vi "gdi32 DeleteObject.vi"(0 "ho":u64, 11 "error in":errorcluster) -> (4 "return value":i32, 15 "error out":errorcluster)   [LabVIEW 2020, in "RemoteVI.lvlib"]
doc: "Deletes a GDI object (bitmap, pen, brush ...) through gdi32.dll DeleteObject (stdcall, called in any thread). It must not be selected into a device context. return value is non-zero on success. When error in carries an error the DLL is not called. Generated by scripts\\Build Win32 Wrappers.vi - do not edit by hand, rebuild it."
uses:
  RemoteVI.lvlib
  gdi32.dll
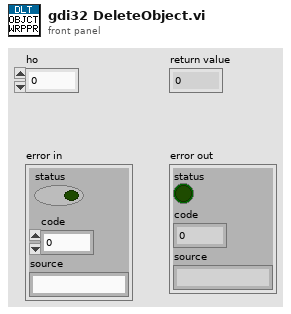
[diagram p1: front panel]
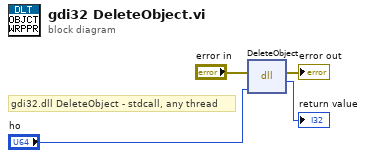
[diagram p0: block diagram]
diagram:
  # "gdi32.dll DeleteObject - stdcall, any thread"
  n1 = dll-call lib="gdi32.dll" fn="DeleteObject"(error in="error in", "ho"="ho") -> (error out=→"error out":errorcluster, →"return value":i32)  [unwired: 3 in, 1 out]
